vi "Actor Core.vi"(8 "error in":errorcluster, 11 "Nested in":refnum<class "AIO_Panel.lvclass">) -> (0 "error out":errorcluster, 3 "Actor out":refnum<class "Actor.lvclass">)   [LabVIEW 2021, in "Simulator-Channel.lvlib" / "AIO_Panel.lvlib" / "AIO_Panel.lvclass"]
doc: "(<B>Filename</B>: Actor Framework.lvlib:Actor.lvclass:Actor Core.vi)\n\nReceives messages to the actor, reacts to them, and initiates any error handling that may shut the actor down.\n\nDescendant classes may override this VI to append parallel tasks for the actor to complete while it handles messages. Overrides use the Call Parent Method node."
uses:
  AIO_Panel.lvclass
  C:/Program Files/National Instruments/LabVIEW 2021/vi.lib/ActorFramework/Actor/Actor.lvclass
  <vilib>/ActorFramework/Actor/Actor.lvclass
  tdef/info.ctl
  <vilib>/ActorFramework/Actor/Actor.lvclass/Actor.ctl
  <vilib>/ActorFramework/Message Enqueuer/Message Enqueuer.lvclass/Message Enqueuer.ctl
  AIO_Panel.lvclass/AIO_Panel.ctl
  DIO_Panel Messages/Update Inputs Msg/Update Inputs Msg.lvclass/Update Inputs Msg.ctl
  <vilib>/ActorFramework/Message Enqueuer/Init from Existing Queue.vi
  <vilib>/ActorFramework/Message Enqueuer/Enqueue.vi
  <vilib>/ActorFramework/Stop Msg/Stop Msg.lvclass
  C:/Program Files/National Instruments/LabVIEW 2021/vi.lib/ActorFramework/Message/Message.lvclass
  DIO_Panel Messages/Update Inputs Msg/Update Inputs Msg.lvclass
  <vilib>/ActorFramework/Message Priority Queue/Priority Enqueue.vi
  <vilib>/ActorFramework/Message Enqueuer/Message Enqueuer.lvclass
panel:
  out "Outputs":T1[](array[typedef])
  in  "Inputs":T1[](array[typedef])
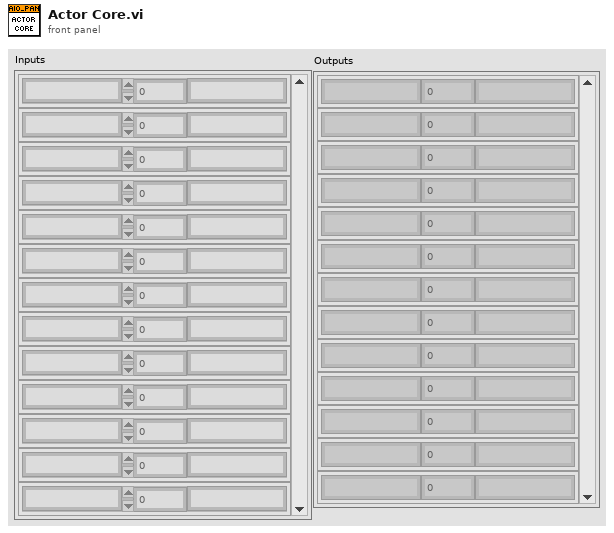
[diagram p1: front panel]
types:
  T1 = typedef "Simulator-Channel.lvlib/AIO_Panel.lvlib/AIO_Panel.lvclass/info.ctl" = cluster{"Name":string, "Numeric":dbl, "Unit":string}
  T2 = cluster{"Stop":refnum<user-event>, "Outputs":refnum<user-event>, "Inputs":refnum<user-event>}
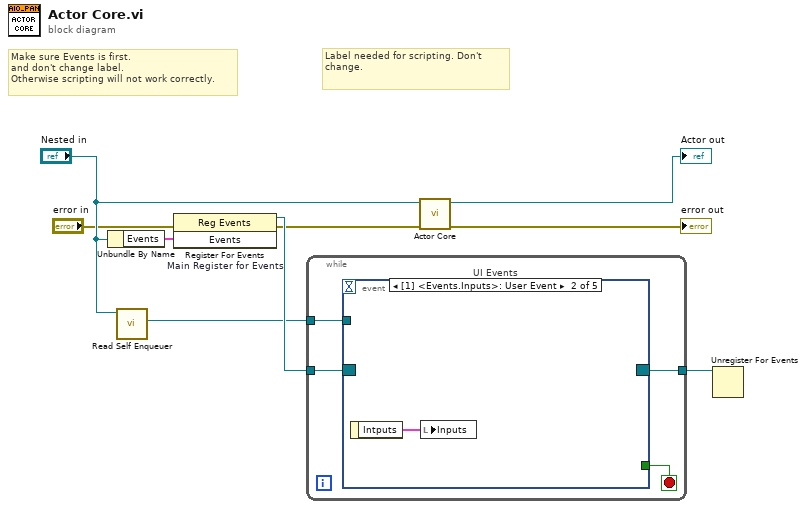
[diagram p0: block diagram]
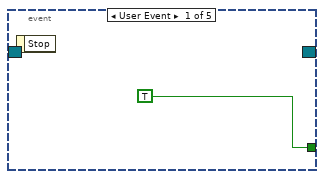
[diagram p2: hidden frame]
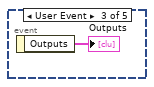
[diagram p3: hidden frame]
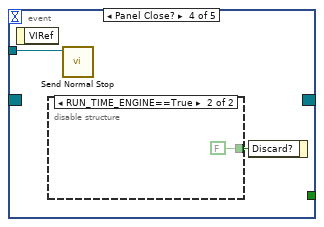
[diagram p4: hidden frame]
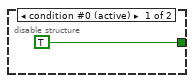
[diagram p5: hidden frame]
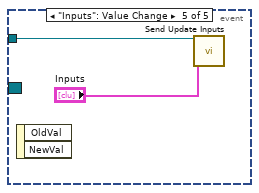
[diagram p6: hidden frame]
diagram:
  # "Label needed for scripting. Don't change."
  # "Make sure Events is first.\nand don't change label.\nOtherwise scripting will not work correctly."
  n1 = Unbundle By Name("Nested in") -> ("Events"=w6:T2)
  n2 = call <vilib>:"Read Self Enqueuer.vi"("Actor"="Nested in") -> ("Self Enqueuer"=w3:refnum<class "Message Enqueuer.lvclass">)  [unwired: 10 in]
  n3 = register-events "Main Register for Events"(error in="error in", w6) -> (reference out=w7:refnum<event-registration>, error out=w1:errorcluster)  [unwired: 1 in]
  n4 = while {
    tunnel: w7 -> [w13]
    tunnel: [w11] -> w5
    tunnel: w3 -> [w10]
    stop <- w12 stop-if-true
    n5 = event "UI Events" shown="[1] <Events.Inputs>: User Event" {
      selector: w13 -> [_ _ _ _ _]
      dyn-events: [_ _ _ _ _] -> w11
      timeout: _ -> [_ _ _ _ _]
      tunnel: [TRUE _ _ _ _] -> w12
      tunnel: w10 -> [_ _ _ w17 w21]
      event User Event {
        n6 = event-data() -> ()  [unwired: 1 in, 1 out]
      }
      event User Event {
        n7 = event-data() -> ("Intputs"=w15:T1[])  [unwired: 1 in]
        n8 = local write "Inputs"(w15) -> ()
      }
      event User Event {
        n9 = event-data() -> ("Outputs"=→"Outputs":T1[])  [unwired: 1 in]
      }
      event Panel Close? {
        n10 = event-data() -> ()  [unwired: 1 in, 1 out]
        n11 = disable-structure shown="RUN_TIME_ENGINE==True" {
          disable-tunnel: [TRUE ("Discard?") FALSE ("Discard?")] -> w18
          frame condition #0 (active) {
          }
          frame condition #1 {
          }
        }
        n12 = call <vilib>:"Send Normal Stop.vi"("Message Enqueuer"=w17) -> ()  [unwired: 10 in, 1 out]
        n13 = event-data("Discard?"=w18) -> ()  [unwired: 1 in, 1 out]
      }
      event "Inputs": Value Change {
        n14 = event-data() -> ()  [unwired: 1 in, 2 out]
        n15 = call "Send Update Inputs.vi"("Inputs"="Inputs", "Message Enqueuer"=w21) -> ()  [unwired: 8 in, 2 out]
      }
    }
  }
  n16 = call-parent "Actor Core.vi"("error in"=w1, "Actor in"="Nested in") -> ("error out"=→"error out":errorcluster, "Actor out"=→"Actor out":refnum<class "Actor.lvclass">)  [unwired: 8 in]
  n17 = Unregister For Events(event registration refnum=w5) -> ()  [unwired: 1 in, 1 out]
